vi "Explore States Dialog.vi"(8 "error in (no error)":errorcluster, 10 "synchronization":refnum<class "synchronization.lvclass">, 11 "Owning VI Details":T1) -> (0 "error out":errorcluster)   [LabVIEW 2020]
uses:
  synchronization/synchronization.lvclass
  synchronization/synchronization.lvclass/synchronization.ctl
  JKI State Machine API/source/JKI SM/JKI SM.lvclass/JKI SM.ctl
  3c27b2d3-2f4c-4225-879f-1b0c2a2f6af0.vi
  <vilib>/Utility/error.llb/Clear Errors.vi
  <userlib>/_OpenG.lib/error/error.llb/Filter Error Codes (Array)__ogtk.vi
  <vilib>/regexp/Match Regular Expression.xnode
  JKI State Machine API/source/JKI SM/JKI SM.lvclass
  <userlib>/_OpenG.lib/error/error.llb/openg_error.lvlib
  <userlib>/_OpenG.lib/string/string.llb/openg_string.lvlib
panel:
  in  "Listbox":i32(listbox)
  in  "OK":bool
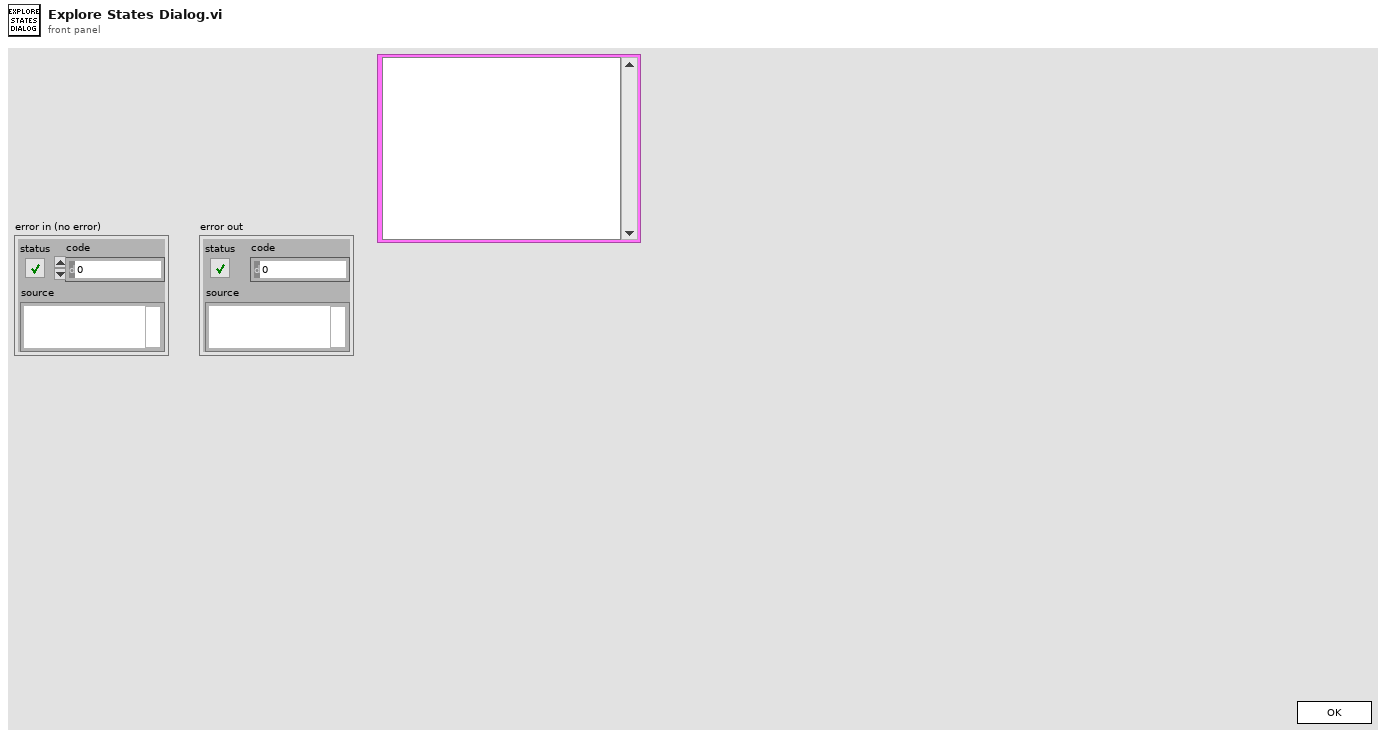
[diagram p1: front panel]
types:
  T1 = cluster{"App.ContextName":string, "VI.Name":string, "Object UID":i32}
  T2 = enum32{"Invalid", "Standard", "Closed", "Hidden", "Minimized", "Maximized"}
  T3 = enum32{"invalid app kind", "Development System", "Run Time System", "Student Edition", "Embedded LabVIEW", "Evaluation", "Custom"}
  T4 = enum32{"Invalid", "Default", "Floating", "Floating/Auto-Hide", "Modal"}
  T5 = cluster{"Core":cluster{"Current VI Reference":refnum<vi>, "Close Panel on Exit?":bool}, "Owning VI":refnum<vi>, "JKI SM out":refnum<class "JKI SM.lvclass">, "States":string[], "StringConstant":refnum<vi>, "Application":refnum<vi>}
  T6 = cluster{"StringConstant":refnum<vi>, "Action":string, "Action":string}
  T7 = typedef "LVPoint32TypeDef.ctl" = cluster{"Horizontal":i32, "Vertical":i32}
  T8 = cluster{"Shift":bool, "Ctrl":bool, "Alt":bool, "Cmd":bool, "Opt":bool}
  T9 = cluster{"StringConstant":refnum<vi>, "Structure":string, "Frame Name":string, "State Call":string, "UID":dbl}[]
  T10 = cluster{"Current VI Reference":refnum<vi>, "Close Panel on Exit?":bool}
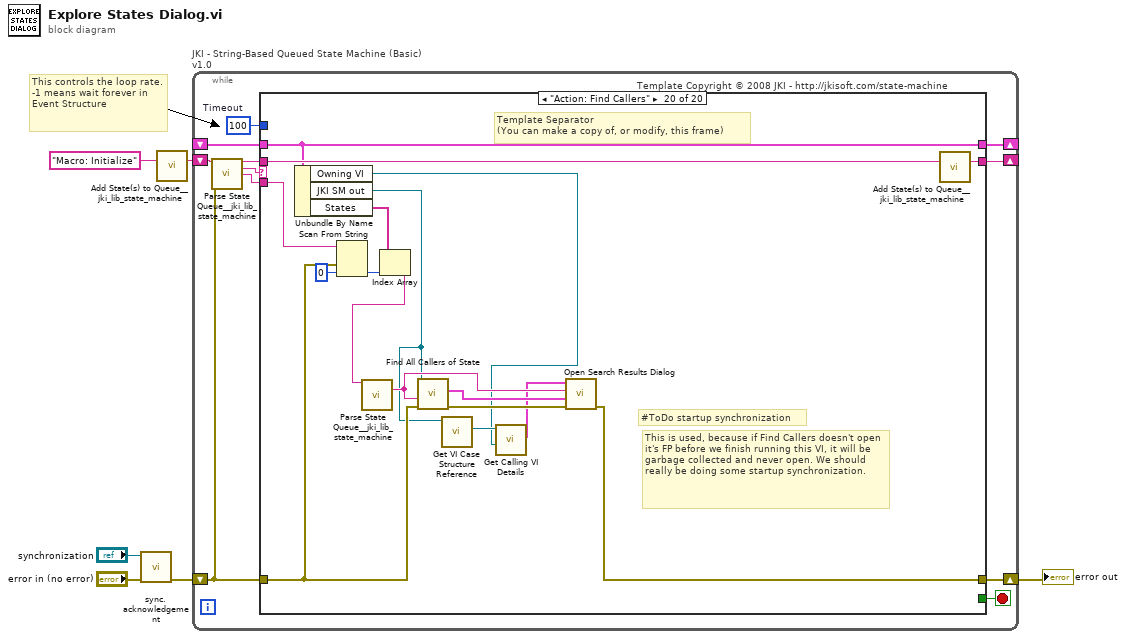
[diagram p0: block diagram]
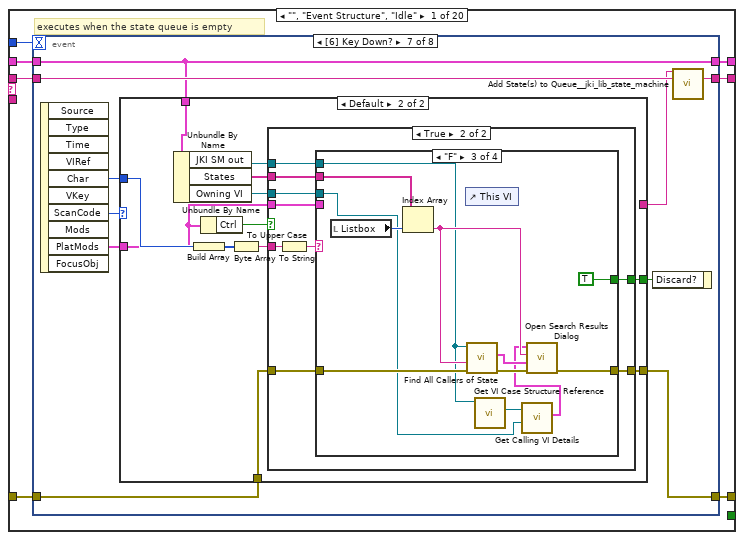
[diagram p2: hidden frame]
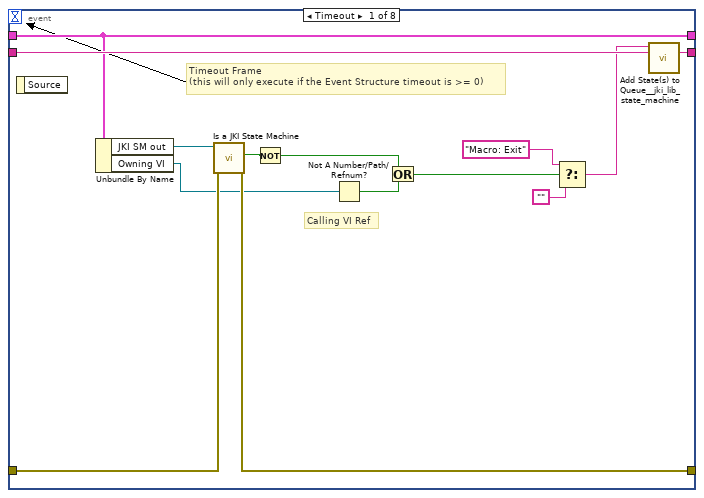
[diagram p3: hidden frame]
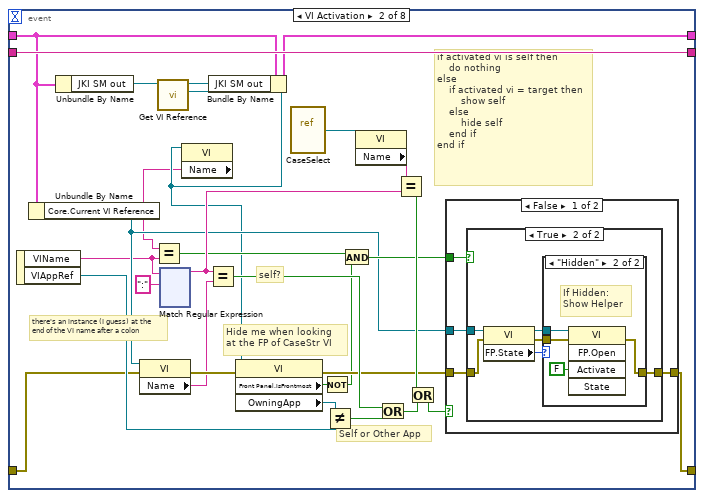
[diagram p4: hidden frame]
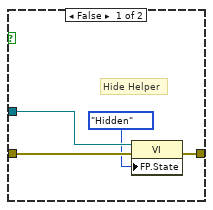
[diagram p5: hidden frame]
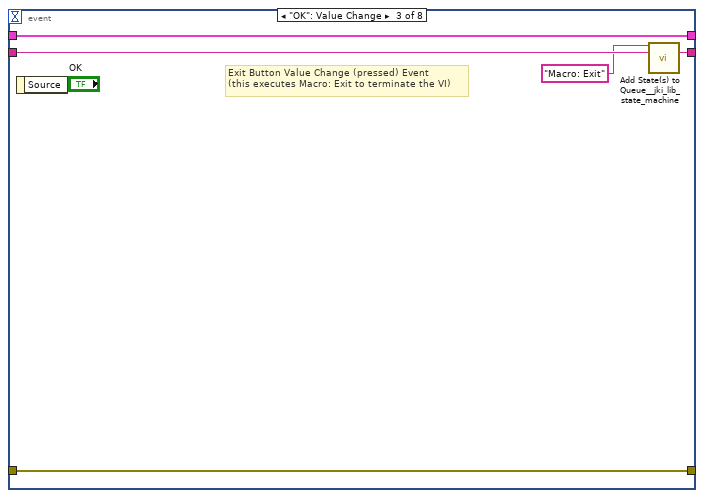
[diagram p8: hidden frame]
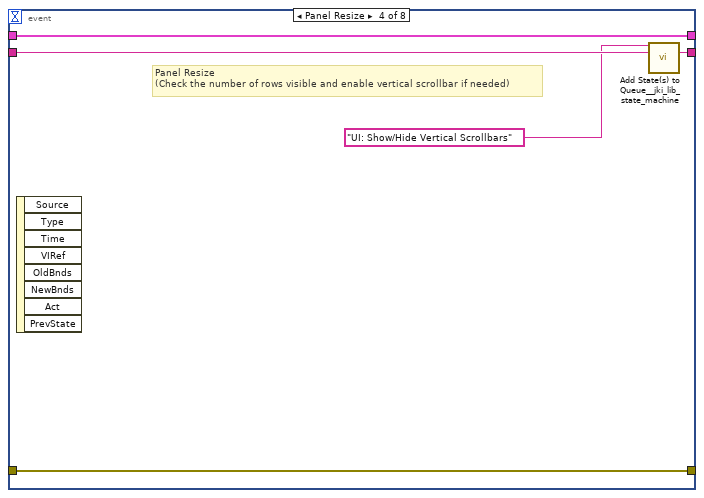
[diagram p9: hidden frame]
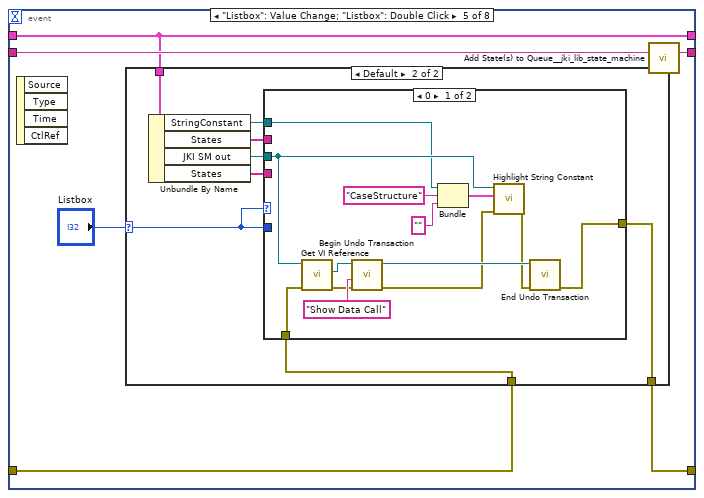
[diagram p10: hidden frame]
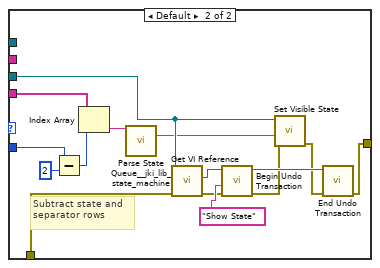
[diagram p12: hidden frame]
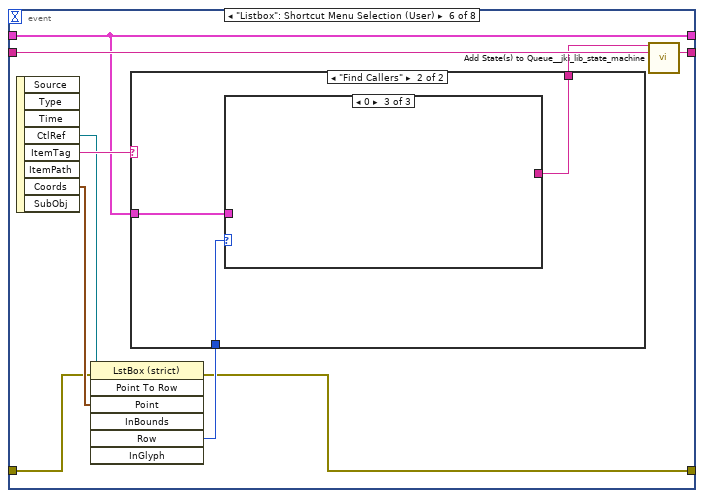
[diagram p13: hidden frame]
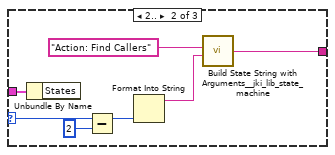
[diagram p16: hidden frame]
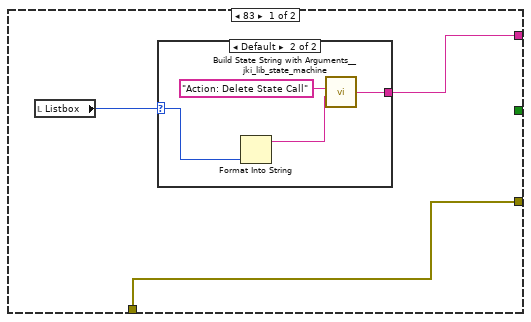
[diagram p17: hidden frame]
diagram:
  # "This controls the loop rate. -1 means wait forever in Event Structure"
  n1 = call "sync.acknowledgement.vi"("error in (no error)"="error in (no error)", "synchronization"="synchronization") -> ("error out"=w1:errorcluster)  [unwired: 9 in]
  n2 = call <vilib>:"Add State(s) to Queue__jki_lib_state_machine.vi"("State(s) in (\"\")"="Macro: Initialize") -> ("States Out"=w6:string)  [unwired: 14 in]
  n3 = while "JKI - String-Based Queued State Machine (Basic) v1.0" {
    shift-right: [w10] -> _
    shift-left: _ -> [w9]
    shift-right: [w13] -> w4
    shift-left: w1 -> [w7]
    shift-right: [w12] -> _
    shift-left: w6 -> [w14]
    stop <- w11 stop-if-true
    w8 = 100  # Timeout
    # "Template Copyright © 2008 JKI - http://jkisoft.com/state-machine"
    n4 = call <vilib>:"Parse State Queue__jki_lib_state_machine.vi"("State Queue"=w14, "Error In (no error)"=w7) -> ("Remaining States"=w16:string, "Current State"=w17:string, "Arguments"=w15:string)  [unwired: 11 in]
    n5 = case shown="\"Action: Find Callers\"" w17 {
      selector: w17 -> [_ _ w362 _ _ _ _ _ _ _ _ _ _ _ _ _ _ _ _ _]
      tunnel: w16 -> [w24 w361 w366 w386 w397 w402 w406 w429 w445 w449 w461 w503 w513 w522 w533 w562 w567 w577 w581 w598]
      tunnel: w15 -> [_ _ _ _ _ _ _ _ _ _ _ _ _ w517 w527 _ _ _ _ w596]
      tunnel: w9 -> [w22 w358 w364 w378 w394 w400 w403 _ w442 w446 w453 w500 w507 w520 w529 w559 w565 w574 w578 w593]
      tunnel: [w21 w359 w368 w373 errorcluster {"status"=FALSE, "code"=0, "source"=""} ("error out") w399 w404 w422 w439 w447 w450 w497 w504 w518 w530 w560 w563 w575 w579 w589] -> w13
      tunnel: w7 -> [w20 w359 w367 w374 w392 w399 w404 w408 w434 w447 w451 w493 w505 w519 w531 w560 w563 w575 w579 w588]
      tunnel: [w23 w360 w365 w385 w396 w401 w405 w428 w444 w448 w460 w502 w512 w521 w532 w561 w566 w576 w580 w597] -> w12
      tunnel: [_ _ _ _ _ TRUE _ _ _ _ _ _ _ _ _ _ _ _ _ _] -> w11
      tunnel: [w19 w358 w364 w384 w394 w400 w403 w427 w442 w446 w453 w476 w507 w520 w529 w559 w565 w574 w578 w593] -> w10
      tunnel: w8 -> [w18 _ _ _ _ _ _ _ _ _ _ _ _ _ _ _ _ _ _ _]
      frame "", "Event Structure", "Idle" {
        # "executes when the state queue is empty"
        n6 = event shown="[6] Key Down?" {
          selector: _ -> [_ _ _ _ _ _ _ _]
          dyn-events: _ -> [_ _ _ _ _ _ _ _]
          timeout: w18 -> [_ _ _ _ _ _ _ _]
          tunnel: w24 -> [w38 w67 w203 w208 w214 w261 w281 w357]
          tunnel: [w37 w67 w202 w207 w213 w260 w280 w356] -> w23
          tunnel: w22 -> [w33 w41 w200 w205 w212 w252 w279 w354]
          tunnel: [w28 w42 w201 w206 w210 w253 w274 w355] -> w21
          tunnel: w20 -> [w29 w43 w201 w206 w211 w255 w275 w355]
          tunnel: [w33 w40 w200 w205 w212 w252 w279 w354] -> w19
          event Timeout {
            # "Calling VI Ref"
            # "Timeout Frame\n(this will only execute if the Event Structure timeout is >= 0)"
            n7 = event-data() -> ()  [unwired: 1 in, 1 out]
            n8 = Unbundle By Name(w33) -> ("JKI SM out"=w32:refnum<class "JKI SM.lvclass">, "Owning VI"=w25:refnum<vi>)
            n9 = call "Is a JKI State Machine.vi"("error in (no error)"=w29, "JKI SM in"=w32) -> ("error out"=w28:errorcluster, "Is a JKI State Machine"=w31:bool)  [unwired: 7 in, 1 out]
            n10 = Not(x=w31) -> (.not. x?=w30:bool)
            n11 = Not A Number/Path/Refnum?(number/path/refnum=w25) -> (NaN/Path/Refnum?=w27:bool)
            n12 = Or(x=w30, y=w27) -> (x .or. y?=w26:bool)
            n13 = Select(t="Macro: Exit", s=w26, f="") -> (s? t:f=w34:string)
            n14 = call <vilib>:"Add State(s) to Queue__jki_lib_state_machine.vi"("State(s) in Front (\"\")"=w34, "State(s) in (\"\")"=w38) -> ("States Out"=w37:string)  [unwired: 13 in]
          }
          event VI Activation {
            # "Self or Other App"
            # "self?"
            # "Hide me when looking\nat the FP of CaseStr VI"
            # "there's an instance (I guess) at the\nend of the VI name after a colon"
            # "if activated vi is self then\n    do nothing\nelse\n    if activated vi = target then\n        show self\n    else\n        hide self\n    end if\nend if"
            n15 = event-data() -> ("VIName"=w45:string, "VIAppRef"=w44:refnum<vi>)  [unwired: 1 in]
            n16 = Unbundle By Name(w41) -> ("Core.Current VI Reference"=w52:refnum<vi>)
            n17 = Unbundle By Name(w41) -> ("JKI SM out"=w48:refnum<class "JKI SM.lvclass">)
            n18 = property class="VI"(reference=w52, error in=w43) -> (error out=w56:errorcluster, "Name"=w51:string)  [unwired: 1 out]
            n19 = call "Get VI Reference.vi"("JKI SM in"=w48) -> ("VI"=w47:refnum<vi>, "JKI SM out"=w39:refnum<class "JKI SM.lvclass">)  [unwired: 8 in, 1 out]
            n20 = xnode "Match Regular Expression"("input string"=w45, "regular expression"=":") -> ("before match"=w63:string)  [unwired: 3 in, 5 out]
            n21 = property class="VI"(reference=w47) -> ("Name"=w46:string)  [unwired: 1 in, 2 out]
            n22 = Equal?(x=w46, y=w45) -> (x = y?=w49:bool)
            n23 = Equal?(x=w63, y=w51) -> (x = y?=w60:bool)
            n24 = Bundle By Name(cluster=w41, "JKI SM out"=w39) -> (w40:T5)
            n25 = property class="VI"(reference=w47, error in=w56) -> (error out=w55:errorcluster, "Front Panel.IsFrontmost"=w53:bool, "OwningApp"=w58:refnum<vi>)  [unwired: 1 out]
            n26 = vi-ref "CaseSelect.vi"() -> (w61:refnum<vi>)
            n27 = Not(x=w53) -> (.not. x?=w54:bool)
            n28 = Not Equal?(x=w58, y=w44) -> (x != y?=w59:bool)
            n29 = And(x=w49, y=w54) -> (x .and. y?=w57:bool)
            n30 = property class="VI"(reference=w61) -> ("Name"=w62:string)  [unwired: 1 in, 2 out]
            n31 = Or(x=w60, y=w59) -> (x .or. y?=w65:bool)
            n32 = Equal?(x=w62, y=w63) -> (x = y?=w64:bool)
            n33 = Or(x=w64, y=w65) -> (x .or. y?=w66:bool)
            n34 = case shown="False" w66 {
              tunnel: w55 -> [w71 w87]
              tunnel: [w69 w87] -> w42
              tunnel: w52 -> [w70 _]
              tunnel: w57 -> [w68 _]
              frame False {
                n35 = case shown="True" w68 {
                  tunnel: w71 -> [w75 w80]
                  tunnel: w70 -> [w74 w81]
                  tunnel: [w73 w78] -> w69
                  frame False {
                    # "Hide Helper"
                    n36 = property class="VI"(reference=w74, error in=w75, "FP.State"=T2."Hidden" ("Front Panel Window:State")) -> (error out=w73:errorcluster)  [unwired: 1 out]
                  }
                  frame True {
                    n37 = property class="VI"(reference=w81, error in=w80) -> (reference out=w77:refnum<vi>, error out=w76:errorcluster, "FP.State"=w79:T2)
                    n38 = case shown="\"Hidden\"" w79 {
                      tunnel: [w82 w86] -> w78
                      tunnel: w77 -> [_ w85]
                      tunnel: w76 -> [w82 w84]
                      frame Default {
                      }
                      frame "Hidden" {
                        # "If Hidden:\nShow Helper"
                        n39 = invoke class="VI" method="FP.Open"(reference=w85, error in=w84, "Activate"=FALSE ("Activate?")) -> (error out=w86:errorcluster)  [unwired: 2 in, 4 out]
                      }
                    }
                  }
                }
              }
              frame True {
              }
            }
          }
          event "OK": Value Change {
            # "Exit Button Value Change (pressed) Event\n(this executes Macro: Exit to terminate the VI)"
            n40 = event-data() -> ()  [unwired: 1 in, 1 out]
            n41 = call <vilib>:"Add State(s) to Queue__jki_lib_state_machine.vi"("State(s) in Front (\"\")"="Macro: Exit", "State(s) in (\"\")"=w203) -> ("States Out"=w202:string)  [unwired: 13 in]
          }
          event Panel Resize {
            # "Panel Resize\n(Check the number of rows visible and enable vertical scrollbar if needed)"
            n42 = event-data() -> ()  [unwired: 1 in, 8 out]
            n43 = call <vilib>:"Add State(s) to Queue__jki_lib_state_machine.vi"("State(s) in Front (\"\")"="UI: Show/Hide Vertical Scrollbars" ("State(s) in Front (\"\")"), "State(s) in (\"\")"=w208) -> ("States Out"=w207:string)  [unwired: 13 in]
          }
          event "Listbox": Value Change; "Listbox": Double Click {
            n44 = event-data() -> ()  [unwired: 1 in, 4 out]
            n45 = case shown="Default" "Listbox" {
              selector: "Listbox" -> [_ w217]
              tunnel: w212 -> [_ w223]
              tunnel: w211 -> [w215 w220]
              tunnel: [w215 w219] -> w210
              frame -1 {
              }
              frame Default {
                n46 = Unbundle By Name(w223) -> ("StringConstant"=w216:refnum<vi>, "States"=w218:string[], "JKI SM out"=w221:refnum<class "JKI SM.lvclass">, "States"=w222:string[])
                n47 = case shown="0" w217 {
                  tunnel: w222 -> [_ w251]
                  tunnel: w221 -> [w235 w244]
                  tunnel: w220 -> [w236 w240]
                  tunnel: w217 -> [_ w249]
                  tunnel: [w234 w241] -> w219
                  tunnel: w218 -> [_ _]
                  tunnel: w216 -> [w233 _]
                  frame 0 {
                    n48 = call "Get VI Reference.vi"("error in (no error)"=w236, "JKI SM in"=w235) -> ("error out"=w231:errorcluster, "VI"=w230:refnum<vi>)  [unwired: 7 in, 1 out]
                    n49 = call "Begin Undo Transaction.vi"("error in (no error)"=w231, "Action"="Show Data Call", "VI in"=w230) -> ("error out"=w227:errorcluster, "VI out"=w229:refnum<vi>)  [unwired: 7 in]
                    n50 = Bundle("StringConstant"=w233, "Action"="CaseStructure", "Action"="") -> (w226:T6)  [unwired: 1 in]
                    n51 = call "Highlight String Constant.vi"("error in (no error)"=w227, "Cluster"=w226, "JKI SM in"=w235) -> ("error out"=w228:errorcluster)  [unwired: 7 in, 1 out]
                    n52 = call "End Undo Transaction.vi"("error in (no error)"=w228, "VI in"=w229) -> ("error out"=w234:errorcluster)  [unwired: 8 in, 1 out]
                  }
                  frame Default {
                    # "Subtract state and separator rows"
                    n53 = Subtract(x=w249, y=2) -> (x-y=w248:i32)
                    n54 = Index Array(array=w251, index=w248) -> (element=w238:string)
                    n55 = call <vilib>:"Parse State Queue__jki_lib_state_machine.vi"("State Queue"=w238) -> ("Current State"=w237:string)  [unwired: 12 in, 2 out]
                    n56 = call "Get VI Reference.vi"("error in (no error)"=w240, "JKI SM in"=w244) -> ("error out"=w246:errorcluster, "VI"=w245:refnum<vi>)  [unwired: 7 in, 1 out]
                    n57 = call "Begin Undo Transaction.vi"("error in (no error)"=w246, "Action"="Show State", "VI in"=w245) -> ("error out"=w239:errorcluster, "VI out"=w243:refnum<vi>)  [unwired: 7 in]
                    n58 = call "Set Visible State.vi"("error in (no error)"=w239, "State Name"=w237, "JKI SM in"=w244) -> ("error out"=w242:errorcluster)  [unwired: 7 in, 1 out]
                    n59 = call "End Undo Transaction.vi"("error in (no error)"=w242, "VI in"=w243) -> ("error out"=w241:errorcluster)  [unwired: 8 in, 1 out]
                  }
                }
              }
            }
            n60 = call <vilib>:"Add State(s) to Queue__jki_lib_state_machine.vi"("State(s) in (\"\")"=w214) -> ("States Out"=w213:string)  [unwired: 14 in]
          }
          event "Listbox": Shortcut Menu Selection (User) {
            n61 = event-data() -> ("CtlRef"=w258:refnum<vi>, "ItemTag"=w259:string, "Coords"=w257:T7)  [unwired: 1 in, 5 out]
            n62 = invoke class="LstBox (strict)" method="Point To Row"(reference=w258, error in=w255, "Point"=w257) -> (error out=w253:errorcluster, "Row"=w256:i32)  [unwired: 4 in, 5 out]
            n63 = case shown="\"Find Callers\"" w259 {
              tunnel: w256 -> [_ w264]
              tunnel: [_ w263] -> w254
              tunnel: w252 -> [_ w262]
              frame Default {
              }
              frame "Find Callers" {
                n64 = case shown="0" w264 {
                  selector: w264 -> [_ w268 _]
                  tunnel: [_ w269 _] -> w263
                  tunnel: w262 -> [_ w265 _]
                  frame -1, Default {
                  }
                  frame 2.. {
                    n65 = Unbundle By Name(w265) -> ()  [unwired: 1 out]
                    n66 = Subtract(x=w268, y=2) -> (x-y=w267:i32)
                    n67 = Format Into String(w267) -> (resulting string=w270:string)  [unwired: 3 in, 1 out]
                    n68 = call <vilib>:"Build State String with Arguments__jki_lib_state_machine.vi"("Arguments (\"\")"=w270, "State"="Action: Find Callers") -> ("State with Arguments"=w269:string)  [unwired: 4 in]
                  }
                  frame 0 {
                  }
                }
              }
            }
            n69 = call <vilib>:"Add State(s) to Queue__jki_lib_state_machine.vi"("State(s) in Front (\"\")"=w254, "State(s) in (\"\")"=w261) -> ("States Out"=w260:string)  [unwired: 13 in]
          }
          event Key Down? {
            n70 = event-data() -> ("Char"=w278:i16, "ScanCode"=w273:i16, "PlatMods"=w277:T8)  [unwired: 1 in, 7 out]
            n71 = case shown="Default" w273 {
              tunnel: w279 -> [_ w300]
              tunnel: w278 -> [_ w298]
              tunnel: w277 -> [_ w295]
              tunnel: [_ w293] -> w276
              tunnel: w275 -> [w283 w291]
              tunnel: [w283 w290] -> w274
              tunnel: [w282 _] -> w272
              frame 83 {
                n72 = local read "Listbox"() -> (w284:i32)
                n73 = case shown="Default" w284 {
                  selector: w284 -> [_ w285]
                  tunnel: [_ w286] -> w282
                  frame -1 {
                  }
                  frame Default {
                    n74 = Format Into String(w285) -> (resulting string=w287:string)  [unwired: 3 in, 1 out]
                    n75 = call <vilib>:"Build State String with Arguments__jki_lib_state_machine.vi"("Arguments (\"\")"=w287, "State"="Action: Delete State Call") -> ("State with Arguments"=w286:string)  [unwired: 4 in]
                  }
                }
              }
              frame Default {
                n76 = Unbundle By Name(w300) -> ("JKI SM out"=w292:refnum<class "JKI SM.lvclass">, "States"=w299:string[], "Owning VI"=w289:refnum<vi>)
                n77 = Build Array(w298) -> (w297:i16[])
                n78 = Unbundle By Name(w295) -> ("Ctrl"=w294:bool)
                n79 = Byte Array To String(unsigned byte array=w297) -> (string=w296:string)
                n80 = case shown="True" w294 {
                  tunnel: w299 -> [_ w310]
                  tunnel: w296 -> [_ w309]
                  tunnel: w295 -> [_ w308]
                  tunnel: [_ w307] -> w293
                  tunnel: w292 -> [_ w305]
                  tunnel: [w301 w304] -> w290
                  tunnel: w291 -> [w301 w303]
                  tunnel: w289 -> [_ w302]
                  frame False {
                  }
                  frame True {
                    n81 = To Upper Case(1:w309) -> (0:w306:string)
                    n82 = case shown="\"F\"" w306 {
                      tunnel: w310 -> [_ w325 w335 _]
                      tunnel: w308 -> [_ w320 _ w344]
                      tunnel: [_ TRUE TRUE TRUE] -> w307
                      tunnel: w305 -> [_ _ w329 w341]
                      tunnel: [w311 w318 w330 w338] -> w304
                      tunnel: w303 -> [w311 w318 w331 w342]
                      tunnel: w302 -> [_ _ w327 _]
                      frame Default {
                      }
                      frame "G" {
                        w313 = 2 ("y")
                        n83 = local read "Listbox"() -> (w315:i32)
                        n84 = Unbundle By Name(w320) -> ("Shift"=w321:bool)
                        n85 = Array Size(array=w325) -> (size(s)=w312:i32)
                        n86 = Subtract(x=w315, y=w313) -> (x-y=w314:i32)
                        n87 = Decrement(x=w314) -> (x-1=w323:i32)
                        n88 = Increment(x=w314) -> (x+1=w324:i32)
                        n89 = Select(t=w323, s=w321, f=w324) -> (s? t:f=w322:i32)
                        n90 = Quotient & Remainder(x=w322, y=w312) -> (x-y*floor(x/y)=w317:i32)  [unwired: 1 out]
                        n91 = Add(x=w317, y=w313) -> (x+y=w316:i32)
                        n92 = property on="Listbox" class="LstBox (strict)"("Val(Sgnl)"=w316) -> ()  [unwired: 2 in, 2 out]
                      }
                      frame "F" {
                        n93 = local read "Listbox"() -> (w336:i32)
                        n94 = Index Array(array=w335, index=w336) -> (element=w334:string)
                        n95 = control-ref of="This VI"() -> ()  [unwired: 1 out]
                        n96 = call "Find All Callers of State.vi"("error in (no error)"=w331, "State Name"=w334, "JKI SM in"=w329) -> ("error out"=w332:errorcluster, "Callers"=w333:T9)  [unwired: 6 in, 1 out]
                        n97 = call "Get VI Case Structure Reference.vi"("JKI SM in"=w329) -> ("Case Structure ref"=w328:refnum<vi>)  [unwired: 8 in, 2 out]
                        n98 = call "Get Calling VI Details.vi"("User VI Ref"=w327, "Affected Items"=w328) -> ("Calling VI Details"=w326:T1)  [unwired: 9 in]
                        n99 = call "Open Search Results Dialog.vi"("error in (no error)"=w332, "Callers"=w333, "State"=w334, "Calling VI Details"=w326) -> ("error out"=w330:errorcluster)  [unwired: 7 in]
                      }
                      frame "Z" {
                        # "Override Ctrl+Z and Ctrl+Shift+Z\n(Handle them here and target the user's VI)"
                        n100 = call "Get VI Reference.vi"("error in (no error)"=w342, "JKI SM in"=w341) -> ("error out"=w339:errorcluster, "VI"=w340:refnum<vi>)  [unwired: 7 in, 1 out]
                        n101 = Unbundle By Name(w344) -> ("Shift"=w343:bool)
                        n102 = case shown="False" w343 {
                          tunnel: w340 -> [w348 w351]
                          tunnel: w339 -> [w346 w350]
                          tunnel: [w347 w349] -> w338
                          frame False {
                            n103 = invoke class="VI" method="Transaction.Undo"(reference=w348, error in=w346) -> (error out=w347:errorcluster)  [unwired: 1 in, 2 out]
                          }
                          frame True {
                            n104 = invoke class="VI" method="Transaction.Redo"(reference=w351, error in=w350) -> (error out=w349:errorcluster)  [unwired: 1 in, 2 out]
                          }
                        }
                      }
                    }
                  }
                }
              }
            }
            n105 = event-data("Discard?"=w276) -> ()  [unwired: 1 in, 1 out]
            n106 = call <vilib>:"Add State(s) to Queue__jki_lib_state_machine.vi"("State(s) in Front (\"\")"=w272, "State(s) in (\"\")"=w281) -> ("States Out"=w280:string)  [unwired: 13 in]
          }
          event Panel Close? {
            # "Discard the event because we'll close the front panel ourselves in Macro: Exit"
            # "Close Panel button (pressed) Event\n(this executes Macro: Exit to terminate the VI)"
            n107 = event-data() -> ()  [unwired: 1 in, 1 out]
            n108 = event-data("Discard?"=TRUE) -> ()  [unwired: 1 in, 1 out]
            n109 = call <vilib>:"Add State(s) to Queue__jki_lib_state_machine.vi"("State(s) in Front (\"\")"="Macro: Exit", "State(s) in (\"\")"=w357) -> ("States Out"=w356:string)  [unwired: 13 in]
          }
        }
      }
      frame "---------- Core ----------" {
        # "Do not put any code in this frame.\n(it is a separator no-op)"
        n110 = call <vilib>:"Add State(s) to Queue__jki_lib_state_machine.vi"("State(s) in (\"\")"=w361) -> ("States Out"=w360:string)  [unwired: 14 in]
      }
      frame Default {
        w371 = 42 items=["No error", "Argument error", "Memory is full", "Out of zone", "End of file", "File already open", "Generic file I/O error", "File not found", "File permission error", "Disk is full", "Duplicate path", "Too many files open", "System feature not enabled", "Resource file not found", "Cannot add resource", "Resource not found", "Image not found", "Image memory error", "Pen does not exist", "Config type invalid", "Config token not found", "Config parse error", "Config memory error", "Bad external code format", "Bad external code offset", "External code not present", "Null window", "Destroy window error", "Null menu", "Print aborted", "Bad print record", "Print driver error", "Windows error during printing", "Memory error during printing", "Print dialog error", "Generic print error", "Invalid device refnum", "Device not found", "Device parameter error", "Device unit error", "Cannot open device", "Device call aborted", "Generic error", "Cancelled by user", "Object ID too low", "Object ID too high", "Object not in heap", "Unknown heap", "Unknown object (invalid DefProc)", "Unknown object (DefProc not in table)", "Message out of range", "Invalid (null) method", "Unknown message", "Manager call not supported", "Bad address", "Network operation in progress", "Network operation timed out", "Connection is busy", "Network attribute not supported", "Network error", "Address in use", "System out of memory", "Connection aborted", "Connection refused", "Not connected", "Already connected", "Connection closed", "Initialization error (interapplication manager)", "Bad occurrence", "Wait on unbound occurrence handler", "Occurrence queue overflow", "Datalog type conflict", "Unused", "Unrecognized type (interapplication manager)", "Memory corrupt", "Failed to make temporary DLL", "Old CIN version", "Drag socket not found", "Failed to load drop-object", "Failed to register OLE object", "Failed to release OLE object", "Format specifier type mismatch", "Unknown format specifier", "Too few format specifiers", "Too many format specifiers", "Scan failed", "Newer CIN version", "Error converting to variant", "Runtime menu error", "Password tampered", "Variant attribute not found", "Incompatible variant data type", "Event data is not available", "Event Store is not present", "Occurrence is not found", "Event Queue is not created", "Event info is not available", "Refnum passed is NULL", "Error retrieving Class GUID", "Error retrieving CoClass GUID", "Error retrieving TypeLib GUID.", "Bad built application magic bytes.", "Specific driver is different from the specific driver associated with the Logical Name.", "There is no session opened to the class driver.", "Max Error", "MAX - Error with config objects", "MAX - Error loading configuration", "MAX - Group not supported"]
        # "Current State"
        # "Do not delete, rename, or modify this frame.\n(this is used to capture unhandled states and typos)"
        # "Handle mistyped state name (developer tool)"
        n111 = Format Into String(format string="Software Exception: Unhandled State \"%s\"." ("message"), error in=w367, w362) -> (resulting string=w370:string, error out=w369:errorcluster)  [unwired: 1 in]
        n112 = call <vilib>:"Error Cluster From Error Code.vi"("show call chain? (False)"=TRUE, "error in (no error)"=w369, "error message (\"\")"=w370, "error code (0)"=w371) -> ("error out"=w368:errorcluster)  [unwired: 5 in]
        n113 = call <vilib>:"Add State(s) to Queue__jki_lib_state_machine.vi"("State(s) in (\"\")"=w366) -> ("States Out"=w365:string)  [unwired: 14 in]
      }
      frame "Initialize Core Data" {
        # "Do not delete, rename, or modify this frame.\n(this is used to determine panel behavior on exit)"
        # "originally closed?"
        # "exe?"
        # "If panel starts closed or is an EXE, then close it when we exit"
        n114 = property class="VI"() -> ("Clone Name"=w376:string)  [unwired: 2 in, 2 out]
        n115 = Open VI Reference(vi path=w376, error in (no error)=w374) -> (vi reference=w375:refnum<vi>, error out=w373:errorcluster)  [unwired: 4 in]
        n116 = property class="VI"() -> ("Front Panel.Open"=w383:bool)  [unwired: 2 in, 2 out]
        n117 = property class="App"() -> ("App.Kind"=w382:T3)  [unwired: 2 in, 2 out]
        n118 = Not(x=w383) -> (.not. x?=w380:bool)
        n119 = Equal?(x=w382, y=T3."Run Time System" ("Application:Kind")) -> (x = y?=w379:bool)
        n120 = Or(x=w380, y=w379) -> (x .or. y?=w377:bool)
        n121 = Bundle By Name(cluster=w378, "Core.Current VI Reference"=w375, "Core.Close Panel on Exit?"=w377) -> (w384:T5)
        n122 = call <vilib>:"Add State(s) to Queue__jki_lib_state_machine.vi"("State(s) in (\"\")"=w386) -> ("States Out"=w385:string)  [unwired: 14 in]
      }
      frame "Error Handler" {
        w393 = i32[] [1026]  # JKI SM VI Invalid Ref
        # "Unhandled Error -- Display it"
        # "Handle any errors here.\nYou can also output any states to clean-up after errors occur"
        # "Clear error"
        n123 = call-poly <userlib>:"Filter Error Codes__ogtk.vi"("Error In"=w392, "Error Codes to Filter"=w393) -> ("Error Out"=w391:errorcluster, "Error Filtered?"=w390:bool)  [unwired: 7 in, 1 out]
        n124 = call <vilib>:"General Error Handler.vi"("error in (no error)"=w391) -> ()  [unwired: 10 in, 5 out]
        n125 = Select(t="Macro: Exit", s=w390, f="") -> (s? t:f=w387:string)
        n126 = call <vilib>:"Add State(s) to Queue__jki_lib_state_machine.vi"("State(s) in Front (\"\")"=w387, "State(s) in (\"\")"=w397) -> ("States Out"=w396:string)  [unwired: 13 in]
      }
      frame "Exit" {
        # "Do not put any code in this frame.\n(No errors that occur here will be handled.)"
        n127 = call <vilib>:"Add State(s) to Queue__jki_lib_state_machine.vi"("State(s) in (\"\")"=w402) -> ("States Out"=w401:string)  [unwired: 14 in]
      }
      frame "---------- Data ----------" {
        # "Do not put any code in this frame.\n(It is a separator no-op. You can make a copy of this frame to create a new Data frame)"
        n128 = call <vilib>:"Add State(s) to Queue__jki_lib_state_machine.vi"("State(s) in (\"\")"=w406) -> ("States Out"=w405:string)  [unwired: 14 in]
      }
      frame "Data: Initialize" {
        w425 = string[] []  # States
        w426 = T10 {"Current VI Reference"=refnum, "Close Panel on Exit?"=FALSE}  # Core
        # "Note from Darren Nattinger regarding menu reference handling in LabVIEW 2024Q3 (and later versions):\nWhen dynamically launching VIs, you must include a delay before creating menu references. LabVIEW will invalidate self-created references if they are generated too soon after VI launch."
        # "do not delete - used by framework"
        # "Data names and types of shift register data are defined by this bundle."
        # "Initialize the shift-register data, here.\n(data names are defined by what you wire into the bundle function)"
        n129 = call "Stall Data Flow.vim"("value in"=w408, "milliseconds to wait"=u32 500) -> ("value out"=w407:errorcluster)  [unwired: 1 out]
        n130 = call "Get Affected Item.vi"("error in (no error)"=w407, "Owning VI Details"="Owning VI Details") -> ("error out"=w414:errorcluster, "GObject"=w416:refnum<vi>, "Owning VI"=w409:refnum<vi>, "Application"=w410:refnum<vi>)  [unwired: 6 in]
        n131 = To More Specific Class(target class=refnum<vi> refnum ("StringConstant"), reference=w416, error in=w414) -> (specific class reference=w415:refnum<vi>, error out=w413:errorcluster)
        n132 = call "Create (From State String Constant).vi"("error in (no error)"=w413, "State String Constant"=w415) -> ("error out"=w418:errorcluster, "JKI SM out"=w419:refnum<class "JKI SM.lvclass">)  [unwired: 6 in, 2 out]
        n133 = property class="StrCnst"(reference=w415, error in=w418) -> (error out=w423:errorcluster, "Text.Text"=w421:string)  [unwired: 1 out]
        n134 = call <userlib>:"Multi-line String to Array__ogtk.vi"("string"=w421) -> ("lines"=w420:string[])
        n135 = Variant To Data(error in=w423, type=w425, Variant=w420) -> (data=w424:string[], error out=w422:errorcluster)
        n136 = Bundle("Core"=w426, "Owning VI"=w409, "JKI SM out"=w419, "States"=w424, "StringConstant"=w415, "Application"=w410) -> (w427:T5)  [unwired: 1 in]
        n137 = call <vilib>:"Add State(s) to Queue__jki_lib_state_machine.vi"("State(s) in (\"\")"=w429) -> ("States Out"=w428:string)  [unwired: 14 in]
      }
      frame "Data: Cleanup" {
        # "Ignore Errors\n(e.g. reference already invalid)"
        # "Cleanup any data and references, here.\n(this is called automatically, by the Macro: Exit)"
        n138 = Unbundle By Name(w442) -> ("Application"=w432:refnum<vi>, "Owning VI"=w431:refnum<vi>, "Core.Current VI Reference"=w443:refnum<vi>, "StringConstant"=w441:refnum<vi>, "JKI SM out"=w435:refnum<class "JKI SM.lvclass">)
        n139 = Close Reference(reference=w443, error in (no error)=w434) -> (error out=w440:errorcluster)
        n140 = Close Reference(reference=w441, error in (no error)=w434) -> (error out=w438:errorcluster)
        n141 = call "Destroy.vi"("error in (no error)"=w434, "JKI SM in"=w435) -> ("error out"=w436:errorcluster)  [unwired: 9 in]
        n142 = call <userlib>:"Clear All Errors__ogtk.vi"("Upsteam Error (optional)"=w434, "Error In"=w436) -> ("Error Out"=w433:errorcluster)  [unwired: 2 in]
        n143 = call <userlib>:"Clear All Errors__ogtk.vi"("Upsteam Error (optional)"=w434, "Error In"=w438) -> ("Error Out"=w437:errorcluster)  [unwired: 2 in]
        n144 = Close Reference(reference=w431) -> (error out=w430:errorcluster)  [unwired: 1 in]
        n145 = Close Reference(reference=w432, error in (no error)=w430) -> ()  [unwired: 1 out]
        n146 = Merge Errors(w440, w437, w433) -> (w439:errorcluster)
        n147 = call <vilib>:"Add State(s) to Queue__jki_lib_state_machine.vi"("State(s) in (\"\")"=w445) -> ("States Out"=w444:string)  [unwired: 14 in]
      }
      frame "---------- UI ----------" {
        # "Do not put any code in this frame.\n(It is a separator no-op. You can make a copy of this frame to create a new UI frame)"
        n148 = call <vilib>:"Add State(s) to Queue__jki_lib_state_machine.vi"("State(s) in (\"\")"=w449) -> ("States Out"=w448:string)  [unwired: 14 in]
      }
      frame "UI: Show/Hide Vertical Scrollbars" {
        # "Add +1 for the Parent Frame and another +1 for the horizontal divider"
        n149 = Unbundle By Name(w453) -> ("States"=w456:string[])
        n150 = Array Size(array=w456) -> (size(s)=w459:i32)
        n151 = property on="Listbox" class="LstBox (strict)"(error in=w451) -> (error out=w452:errorcluster, "Number of Rows"=w458:u32)  [unwired: 1 in, 1 out]
        n152 = Increment(x=w459) -> (x+1=w455:i32)
        n153 = Increment(x=w455) -> (x+1=w454:i32)
        n154 = Greater Or Equal?(x=w454, y=w458) -> (x >= y?=w457:bool)
        n155 = property on="Listbox" class="LstBox (strict)"(error in=w452, "Scrollbar Visible"=w457) -> (error out=w450:errorcluster)  [unwired: 1 in, 1 out]
        n156 = call <vilib>:"Add State(s) to Queue__jki_lib_state_machine.vi"("State(s) in (\"\")"=w461) -> ("States Out"=w460:string)  [unwired: 14 in]
      }
      frame "UI: Initialize" {
        # "Initialize the User Interface, here.\n(this is called automatically, by the Macro: Init)"
        n157 = Unbundle By Name(w500) -> ("Core.Current VI Reference"=w501:refnum<vi>, "States"=w472:string[], "JKI SM out"=w498:refnum<class "JKI SM.lvclass">, "StringConstant"=w499:refnum<vi>)
        n158 = property class="StrCnst"(reference=w499, error in=w493) -> (error out=w492:errorcluster, "Label.Text"=w489:string)  [unwired: 1 out]
        n159 = Empty String/Path?(string/path=w489) -> (empty?=w496:bool)
        n160 = call "Get State String Info.vi"("error in (no error)"=w492, "GObj Refnum in"=w499, "JKI SM in"=w498) -> ("error out"=w497:errorcluster, "Frame Name"=w491:string, "Structure"=w483:string, "JKI SM out"=w462:refnum<class "JKI SM.lvclass">)  [unwired: 5 in]
        n161 = Not(x=w496) -> (.not. x?=w494:bool)
        n162 = Not Equal?(x=w491, y=w489) -> (x != y?=w495:bool)
        n163 = Equal?(x="EventStructure", y=w483) -> (x = y?=w484:bool)
        n164 = And(x=w495, y=w494) -> (x .and. y?=w490:bool)
        n165 = Build Array(w489) -> (w488:string[])
        n166 = Build Array(w483) -> (w482:string[])
        n167 = Select(t=w488, s=w490, f=string[] []) -> (s? t:f=w487:string[])
        n168 = Select(t=w482, s=w484, f=string[] []) -> (s? t:f=w480:string[])
        n169 = Build Array (concatenate)(w480, w491, w487) -> (w479:string[])
        n170 = call <userlib>:"1D Array to String__ogtk.vi"("delimiter (Tab)"=": ", "Array of Strings"=w479) -> ("delimited string"=w475:string)  [unwired: 9 in]
        n171 = Format Into String(format string="Back to %s", w475) -> (resulting string=w473:string)  [unwired: 2 in, 1 out]
        n172 = property class="VI"(reference=w501, "Front Panel.Title"="String Constant" ("format string")) -> ()  [unwired: 1 in, 2 out]
        n173 = Build Array (concatenate)(w473, "" ("format string"), w472) -> (w468:string[])
        n174 = Bundle By Name(cluster=w500, "JKI SM out"=w462) -> (w476:T5)
        n175 = property on="Listbox" class="LstBox (strict)"("Item Names"=w468, "Value"=-1 ("Listbox")) -> (error out=w467:errorcluster, "Item Symbols"=w466:i32[])  [unwired: 2 in, 1 out]
        n176 = Replace Array Subset(array=w466, new element=-1 ("new element/subarray"), index=1) -> (w465:i32[])
        n177 = property on="Listbox" class="LstBox (strict)"(error in=w467, "Item Symbols"=w465) -> ()  [unwired: 1 in, 2 out]
        n178 = call <vilib>:"Add State(s) to Queue__jki_lib_state_machine.vi"("State(s) in Front (\"\")"="UI: Show/Hide Vertical Scrollbars" ("State(s) in Front (\"\")"), "State(s) in (\"\")"=w503) -> ("States Out"=w502:string)  [unwired: 13 in]
      }
      frame "UI: Pre-Test for 0 or 1 Items" {
        n179 = Unbundle By Name(w507) -> ("JKI SM out"=w508:refnum<class "JKI SM.lvclass">, "JKI SM out"=w510:refnum<class "JKI SM.lvclass">, "States"=w509:string[])
        n180 = Array Size(array=w509) -> (size(s)=w511:i32)
        n181 = case shown="Default" w511 {
          tunnel: w510 -> [_ _]
          tunnel: [_ "Macro: Exit"] -> w506
          tunnel: w509 -> [_ _]
          tunnel: w508 -> [_ _]
          tunnel: w505 -> [w514 w515]
          tunnel: [w514 w515] -> w504
          frame Default {
          }
          frame 0 {
          }
        }
        n182 = call <vilib>:"Add State(s) to Queue__jki_lib_state_machine.vi"("State(s) in Front (\"\")"=w506, "State(s) in (\"\")"=w513) -> ("States Out"=w512:string)  [unwired: 13 in]
      }
      frame "UI: Cursor Set" {
        # "Argument"
        # "Set and Unset Cursor Busy.\n(Usage: \"UI: Cursor Set >> Busy|Idle\")"
        n183 = case shown="\"Idle\", Default" w517 {
          tunnel: w519 -> [w524 w526]
          tunnel: [w523 w525] -> w518
          frame "Idle", Default {
            n184 = call <vilib>:"Unset Busy.vi"("error in (no error)"=w524) -> ("error out"=w523:errorcluster)  [unwired: 10 in]
          }
          frame "Busy" {
            n185 = call <vilib>:"Set Busy.vi"("error in (no error)"=w526) -> ("error out"=w525:errorcluster)  [unwired: 9 in, 1 out]
          }
        }
        n186 = call <vilib>:"Add State(s) to Queue__jki_lib_state_machine.vi"("State(s) in (\"\")"=w522) -> ("States Out"=w521:string)  [unwired: 14 in]
      }
      frame "UI: Front Panel State" {
        # "Argument"
        # "Set Front Panel Open or Closed\n(Usage: \"UI: Front Panel State >> Open|Close\")"
        n187 = Unbundle By Name(w529) -> ("Core.Current VI Reference"=w528:refnum<vi>)
        n188 = case shown="\"Open\", Default" w527 {
          tunnel: w531 -> [w537 w553]
          tunnel: [w539 w554] -> w530
          tunnel: w528 -> [w538 w551]
          frame "Open", Default {
            n189 = property class="VI"(reference=w538, error in=w537) -> (reference out=w535:refnum<vi>, error out=w536:errorcluster, "Front Panel.Open"=w534:bool)
            n190 = case shown="False" w534 {
              tunnel: [w542 w548] -> w539
              tunnel: w536 -> [w545 w548]
              tunnel: w535 -> [w544 _]
              frame False {
                # "Setting Floatin here, instead of VI Properties allows the VI to accept keyboard input immediately after openning. (setting it in VI Properties was causing a bug where it wouldn't receive keyboard input until clicking on the VI)"
                n191 = invoke class="VI" method="FP.Open"(reference=w544, error in=w545, "Activate"=TRUE, "State"=T2."Standard") -> (reference out=w541:refnum<vi>, error out=w543:errorcluster)  [unwired: 1 in, 3 out]
                n192 = property class="VI"(reference=w541, error in=w543, "FP.Behavior"=T4."Floating" ("Front Panel Window:Behavior")) -> (error out=w542:errorcluster)  [unwired: 1 out]
              }
              frame True {
              }
            }
          }
          frame "Close" {
            n193 = property class="VI"(reference=w551, error in=w553) -> (reference out=w550:refnum<vi>, error out=w552:errorcluster, "Front Panel.Open"=w549:bool)
            n194 = case shown="True" w549 {
              tunnel: [w555 w558] -> w554
              tunnel: w552 -> [w555 w557]
              tunnel: w550 -> [_ w556]
              frame False {
              }
              frame True {
                n195 = invoke class="VI" method="FP.Close"(reference=w556, error in=w557) -> (error out=w558:errorcluster)  [unwired: 1 in, 2 out]
              }
            }
          }
        }
        n196 = call <vilib>:"Add State(s) to Queue__jki_lib_state_machine.vi"("State(s) in (\"\")"=w533) -> ("States Out"=w532:string)  [unwired: 14 in]
      }
      frame "---------- Macro ----------" {
        # "Do not put any code in this frame.\n(It is a separator no-op. You can make a copy of this frame to create a new Macro frame)"
        n197 = call <vilib>:"Add State(s) to Queue__jki_lib_state_machine.vi"("State(s) in (\"\")"=w562) -> ("States Out"=w561:string)  [unwired: 14 in]
      }
      frame "Macro: Initialize" {
        w564 = "Data: Initialize\nInitialize Core Data\nUI: Pre-Test for 0 or 1 Items\nUI: Initialize\nUI: Front Panel State >> Open"  # Data: Initialize Initialize Core Data UI: Pre-Test for 0 or 1 Items UI: Initialize UI: Front Panel State >> Open
        # "Initialization Macro\n(This is called once, when the VI starts)"
        n198 = call <vilib>:"Add State(s) to Queue__jki_lib_state_machine.vi"("State(s) in Front (\"\")"=w564, "State(s) in (\"\")"=w567) -> ("States Out"=w566:string)  [unwired: 13 in]
      }
      frame "Macro: Exit" {
        # "Exit Macro\n(This is called once, when the VI exits)"
        n199 = Unbundle By Name(w574) -> ("Core.Close Panel on Exit?"=w573:bool)
        n200 = Select(t="UI: Front Panel State >> Close", s=w573, f="") -> (s? t:f=w570:string)
        n201 = call <vilib>:"Add State(s) to Queue__jki_lib_state_machine.vi"("State(s) in (\"\")"=w570, "State(s) at Back (\"\")"="Data: Cleanup\nExit") -> ("States Out"=w568:string)  [unwired: 13 in]
        n202 = call <vilib>:"Add State(s) to Queue__jki_lib_state_machine.vi"("State(s) in Front (\"\")"=w568, "State(s) in (\"\")"=w577) -> ("States Out"=w576:string)  [unwired: 13 in]
      }
      frame "---------- Action ----------" {
        # "Template Separator\n(You can make a copy of, or modify, this frame)"
        n203 = call <vilib>:"Add State(s) to Queue__jki_lib_state_machine.vi"("State(s) in (\"\")"=w581) -> ("States Out"=w580:string)  [unwired: 14 in]
      }
      frame "Action: Find Callers" {
        # "#ToDo startup synchronization"
        # "This is used, because if Find Callers doesn't open it's FP before we finish running this VI, it will be garbage collected and never open. We should really be doing some startup synchronization."
        # "Template Separator\n(You can make a copy of, or modify, this frame)"
        n204 = Unbundle By Name(w593) -> ("Owning VI"=w582:refnum<vi>, "JKI SM out"=w584:refnum<class "JKI SM.lvclass">, "States"=w592:string[])
        n205 = Scan From String(input string=w596, error in=w588, default 1=0 ("default value 1")) -> (output 1=w594:i32)  [unwired: 2 in, 3 out]
        n206 = Index Array(array=w592, index=w594) -> (element=w587:string)
        n207 = call <vilib>:"Parse State Queue__jki_lib_state_machine.vi"("State Queue"=w587) -> ("Current State"=w586:string)  [unwired: 12 in, 2 out]
        n208 = call "Find All Callers of State.vi"("error in (no error)"=w588, "State Name"=w586, "JKI SM in"=w584) -> ("error out"=w590:errorcluster, "Callers"=w591:T9)  [unwired: 6 in, 1 out]
        n209 = call "Get VI Case Structure Reference.vi"("JKI SM in"=w584) -> ("Case Structure ref"=w583:refnum<vi>)  [unwired: 8 in, 2 out]
        n210 = call "Get Calling VI Details.vi"("User VI Ref"=w582, "Affected Items"=w583) -> ("Calling VI Details"=w585:T1)  [unwired: 9 in]
        n211 = call "Open Search Results Dialog.vi"("error in (no error)"=w590, "Callers"=w591, "State"=w586, "Calling VI Details"=w585) -> ("error out"=w589:errorcluster)  [unwired: 7 in]
        n212 = call <vilib>:"Add State(s) to Queue__jki_lib_state_machine.vi"("State(s) in (\"\")"=w598) -> ("States Out"=w597:string)  [unwired: 14 in]
      }
    }
  }
  "error out" <- w4
